vi "Glimpse Image Display Controller.vi"() -> ()   [LabVIEW 2015]
doc: "This widget allows the user to separately adjust the properties of mulltiple, independently displayed image windows. The controller is a stand-alone VI that can run in a separate thread from the program that is producing the images, so that the image display settings can be adjusted whilst other things (e.g., data acquisition) are occurring simultaneously."
uses:
  Image to Display event.ctt
  <vilib>/vision/Image Controls.llb/IMAQ Image.ctl
  GLIMPSE Globals.vi
panel:
  in  "to window":i8=9 min=2 max=9 step=1
  in  "Snapshot":bool
  in  "Presets":T1(array[cluster])=[{"Mem"=FALSE, "Black"=-32500.0, "White"=-25000.0, "Recall"=FALSE}]
  in  "Keep this in corner?":bool=TRUE
  in  "Autosize M":bool
  in  "Autoposition M":bool
  in  "Autoscale M":bool
  in  "Zoom +":bool
  in  "Zoom -":bool
  out "In use":bool
  in  "Auto size":bool
  in  "Auto position":bool
  in  "Autoscale":bool
  out "Window Title":string
  in  "Control image window #":u8(slide)=1 max=1 step=1 scale=0.0..1.0
  out "error out":errorcluster
  out "Black/White Levels temp":cluster{ext, ext}(slide)={1.0, 65535.0} scale=-32767.0..327567.0
  in  "Black/White Levels":cluster{ext, ext}(slide)={1.0, 65535.0} scale=-32767.0..327567.0
  in  "Stop":bool
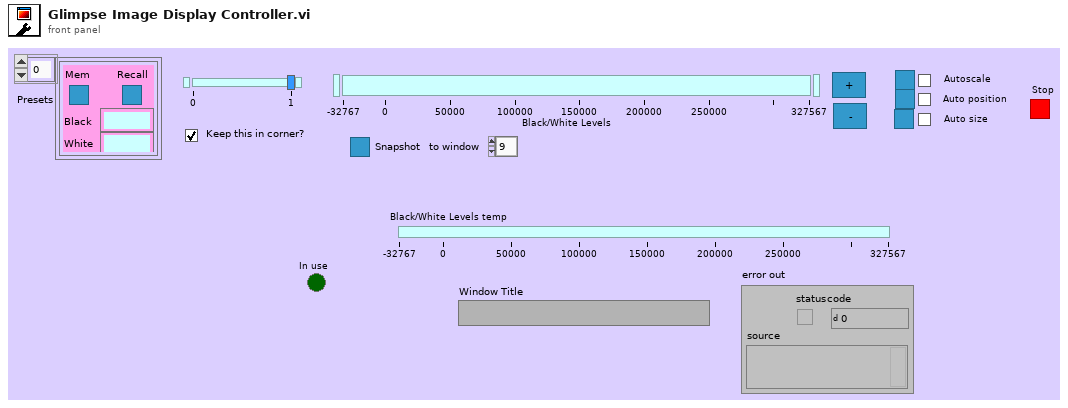
[diagram p1: front panel]
types:
  T1 = cluster{"Mem":bool, "Black":ext, "White":ext, "Recall":bool}[]
  T2 = typedef "Image Type" = u32
  T3 = typedef "IMAQ Image.ctl" = refnum<image>
  T4 = cluster{"Image Type":T2, "Image":T3, "Initialized?":bool, "Window Title":string, "Auto resize?":bool, "Auto position?":bool, "Autoscale?":bool, "Black/White Levels":cluster{ext, ext}, "Scale Min":ext, "Scale Max":ext}
  T5 = typedef "LVRectTypeDef.ctl" = cluster{"Left":i16, "Top":i16, "Right":i16, "Bottom":i16}
  T6 = typedef "Image to Display event.ctt" = cluster{"Image":T3, "Window Title":string, "Window Number":i32, "Image Type":T2, "Quit display controller?":bool}
  T7 = cluster{"Image Type":T2, "Image":T3, "Initialized?":bool, "Window Title":string, "Auto resize?":bool, "Auto position?":bool, "Autoscale?":bool, "Black/White Levels":cluster{ext, ext}, "Scale Min":ext, "Scale Max":ext}[]
  T8 = cluster{"Mem":bool, "Black":ext, "White":ext, "Recall":bool}
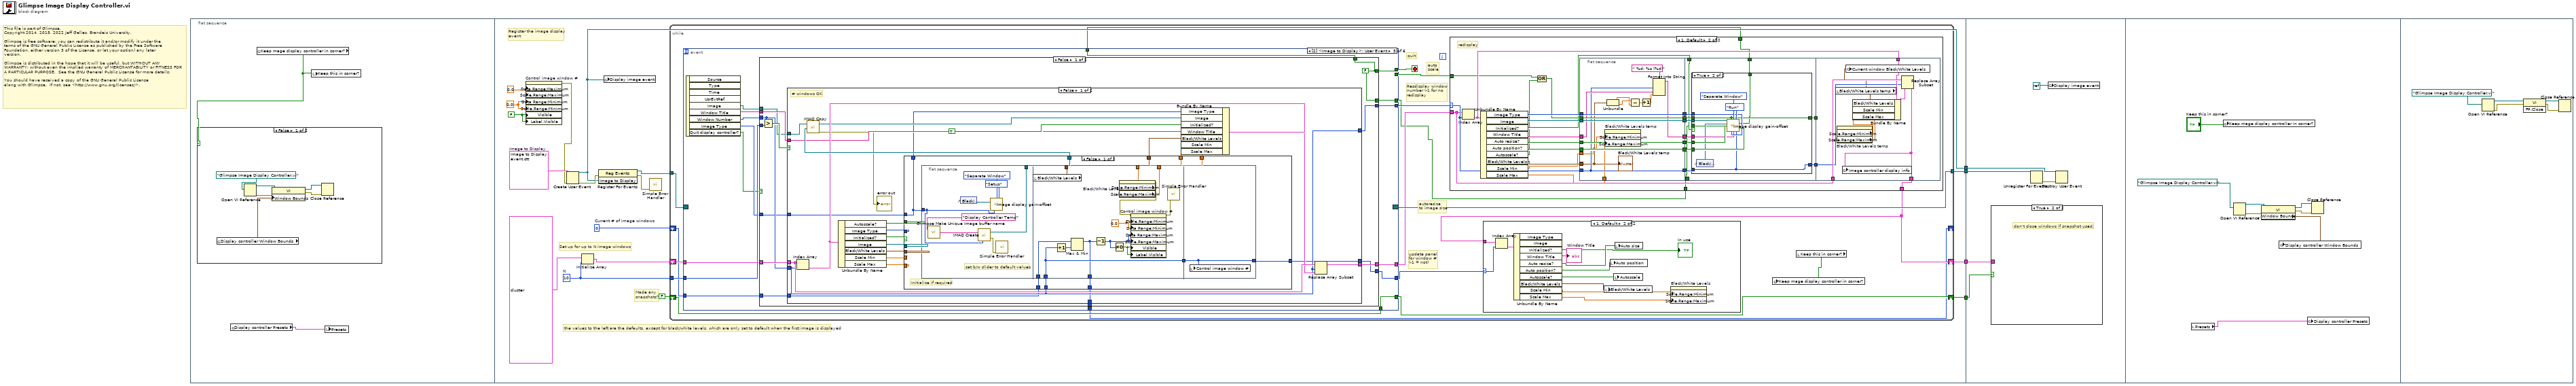
[diagram p0: block diagram]
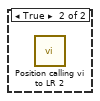
[diagram p2: hidden frame]
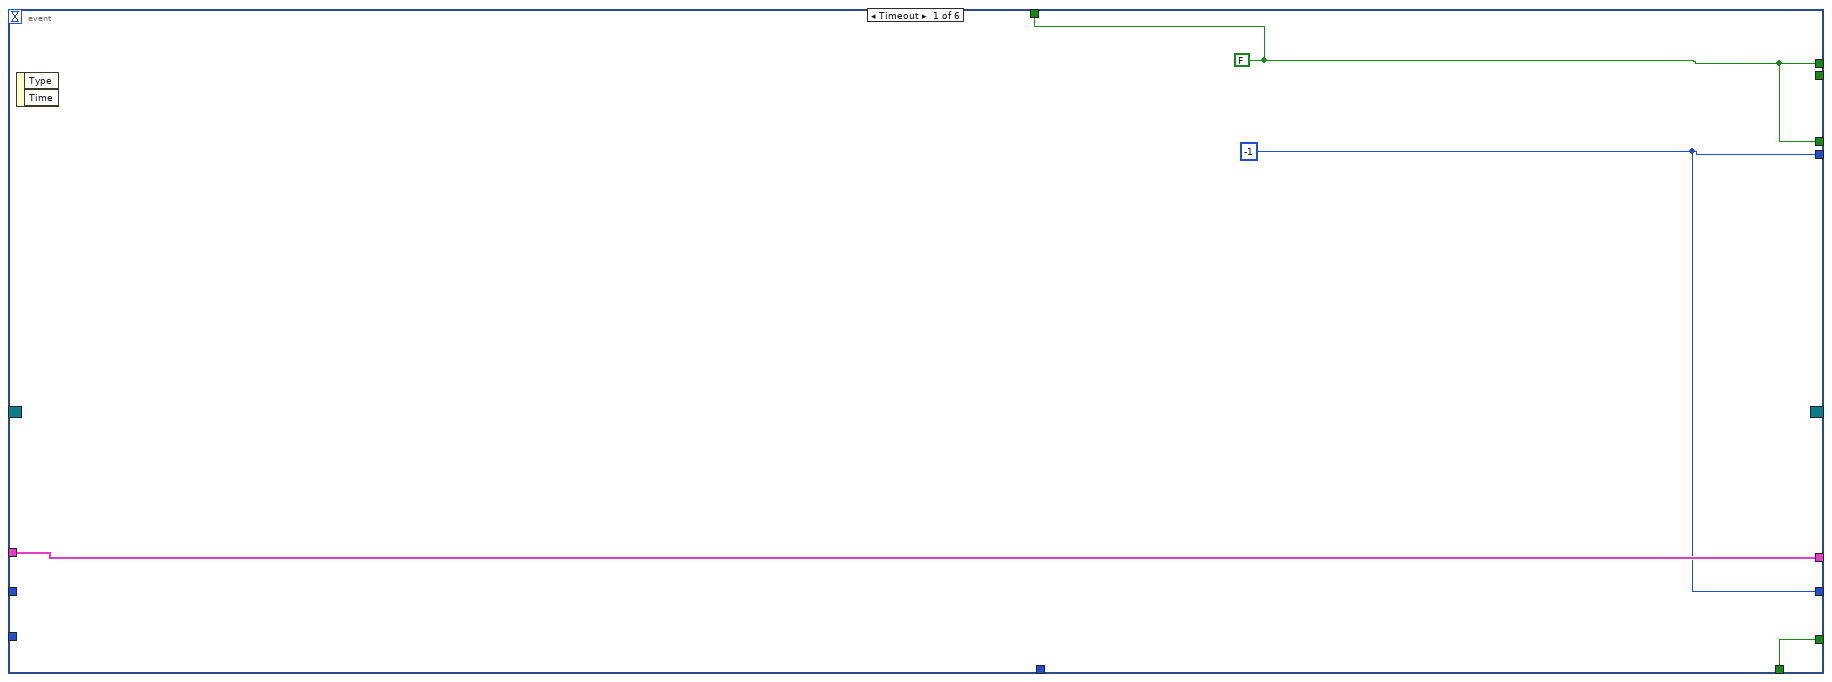
[diagram p6: hidden frame]
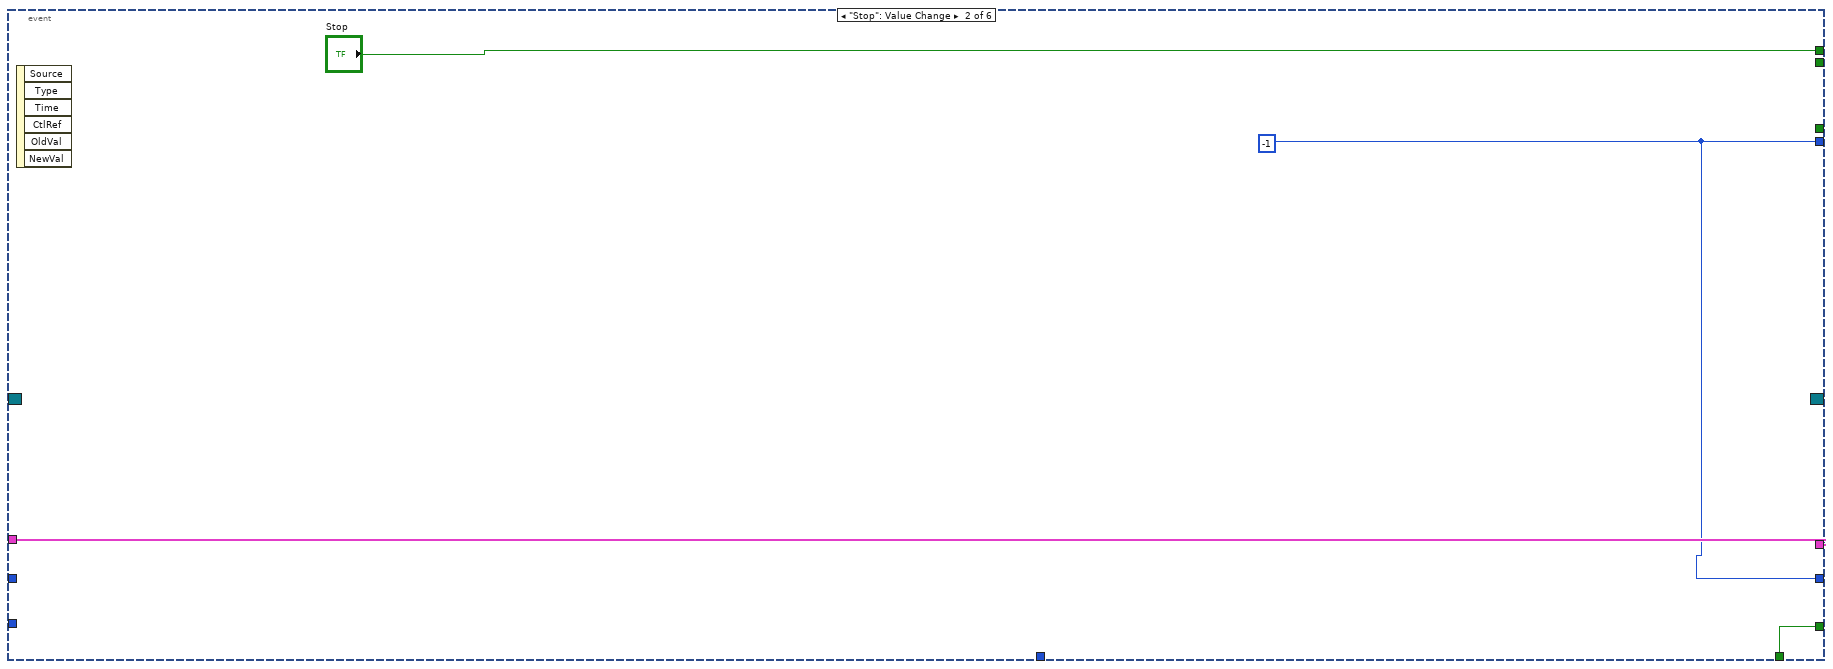
[diagram p7: hidden frame]
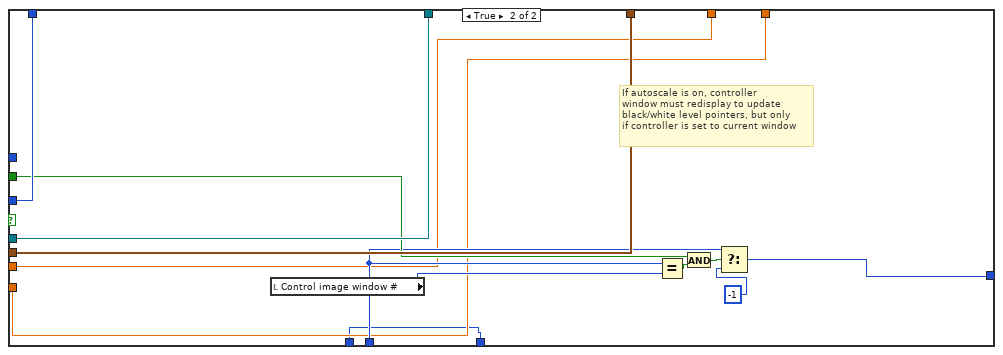
[diagram p8: hidden frame]
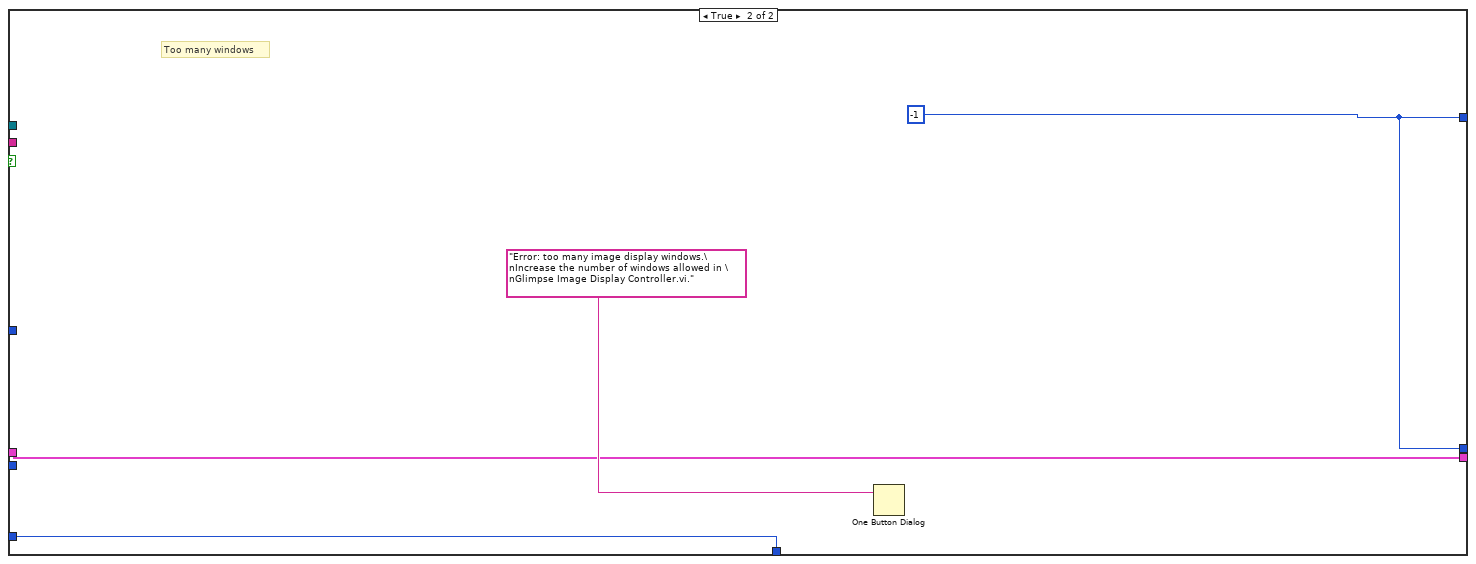
[diagram p9: hidden frame]
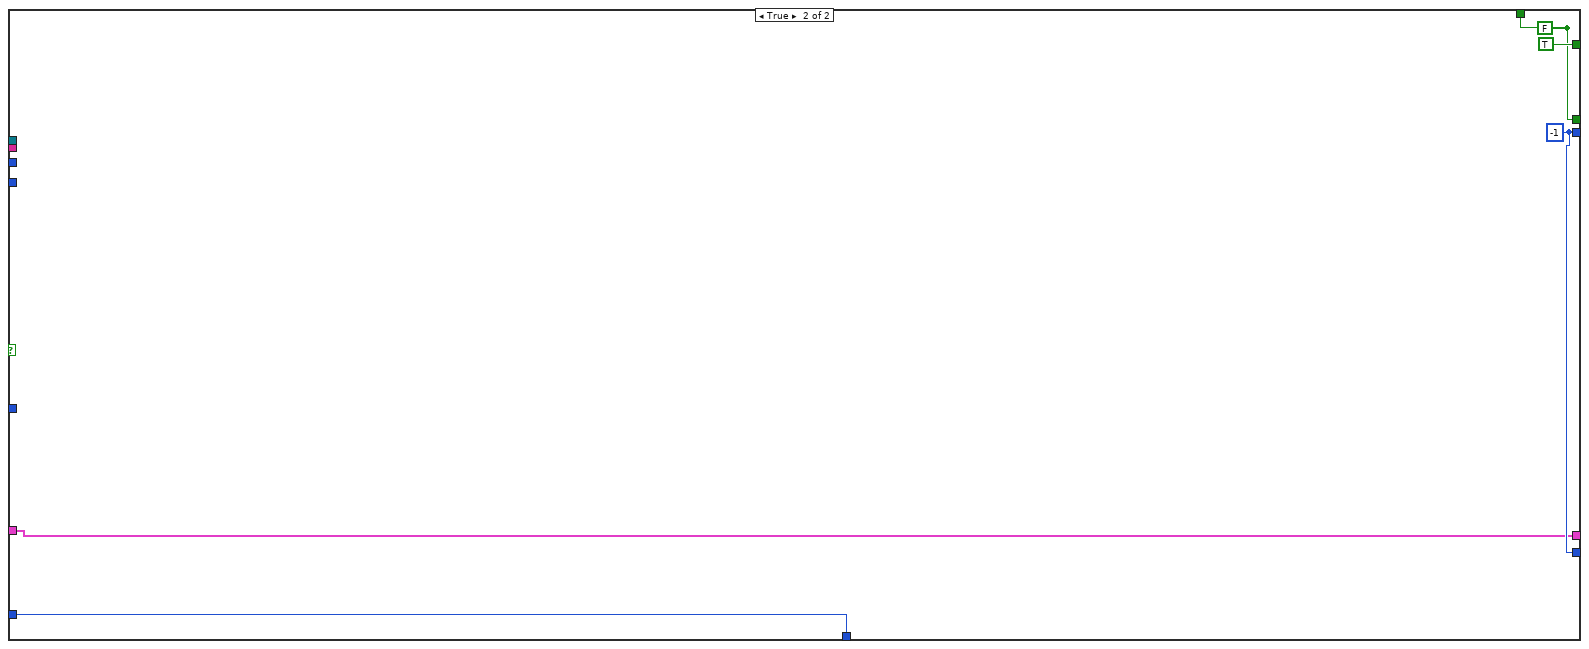
[diagram p10: hidden frame]
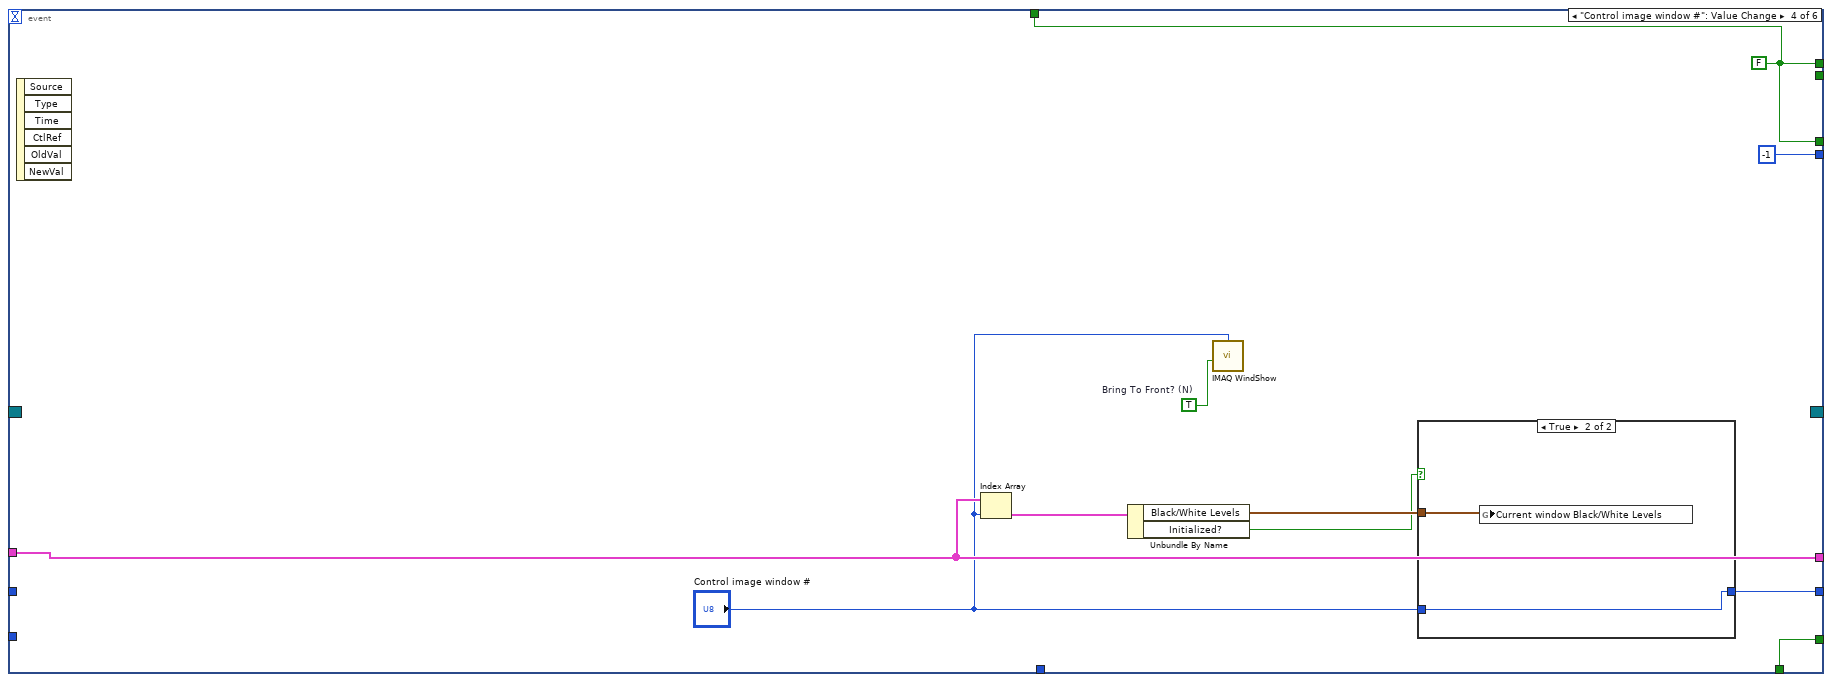
[diagram p11: hidden frame]
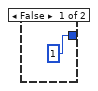
[diagram p12: hidden frame]
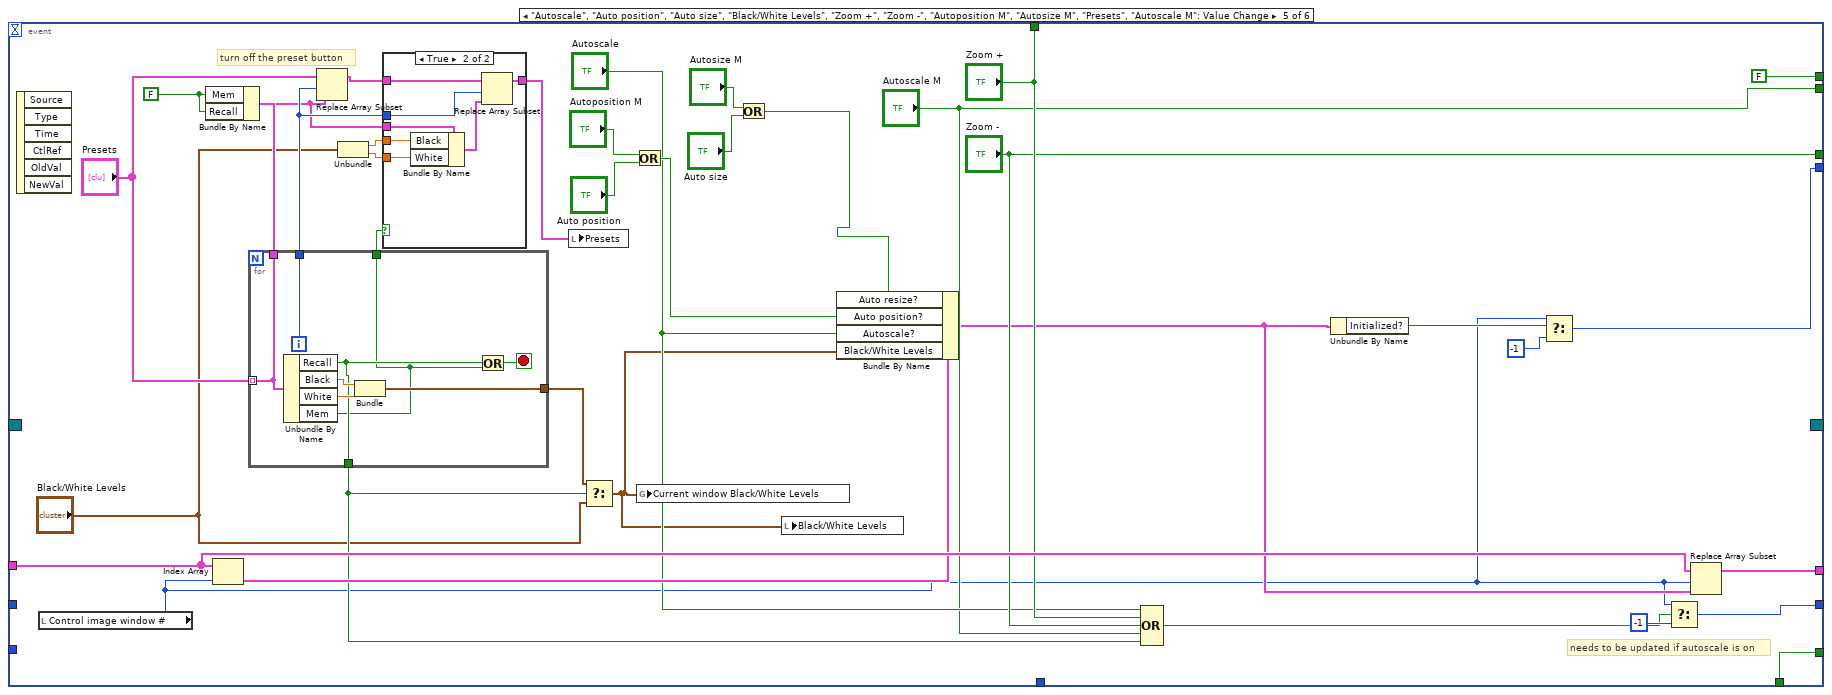
[diagram p13: hidden frame]
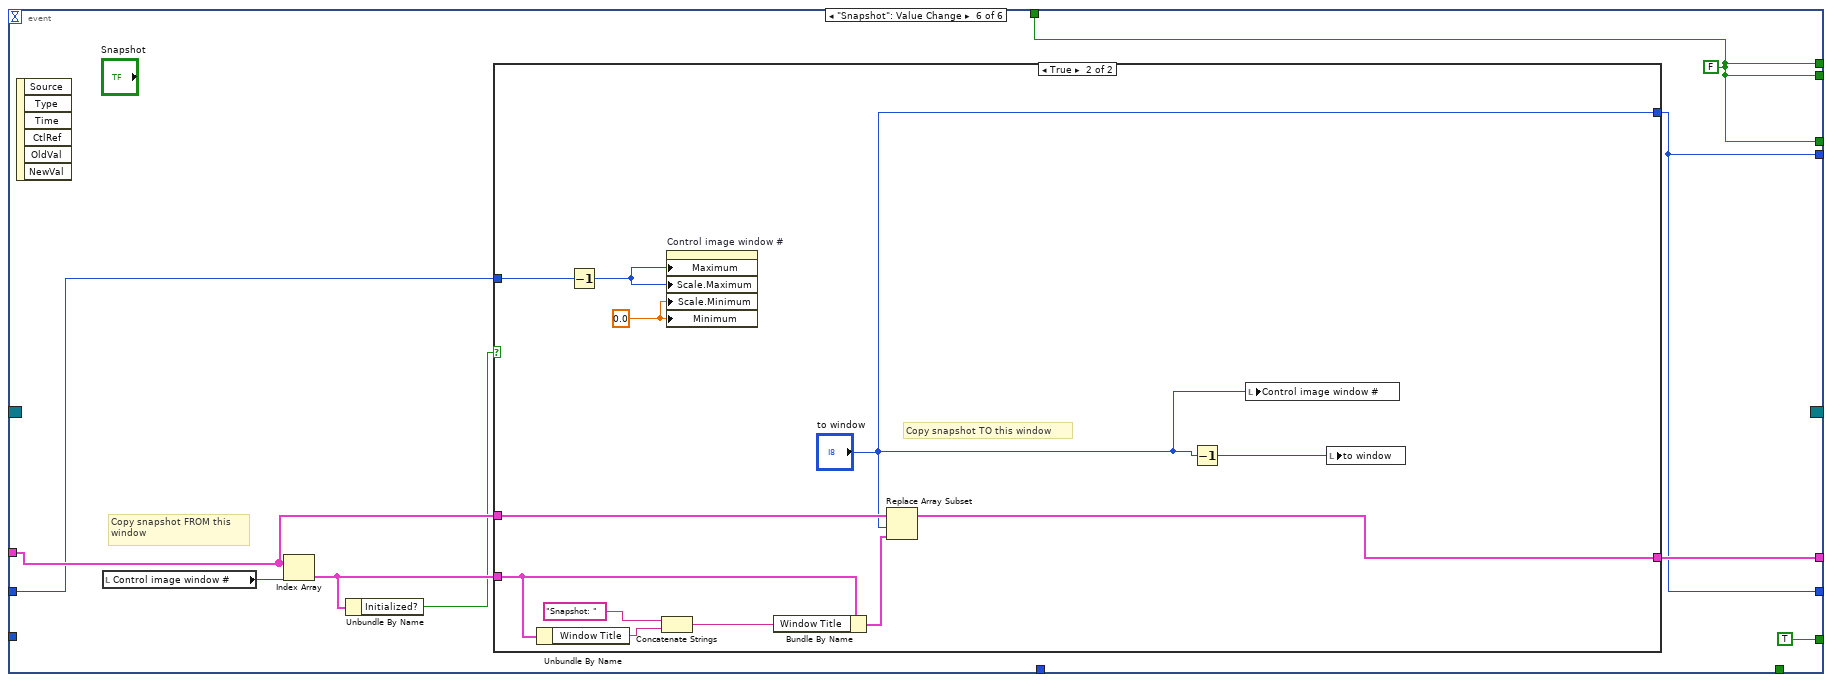
[diagram p15: hidden frame]
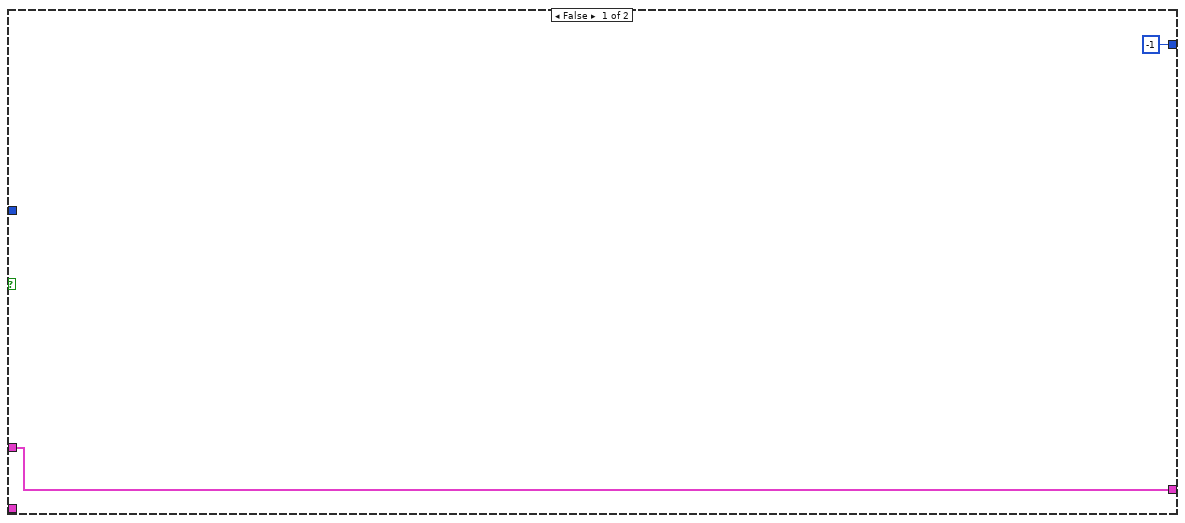
[diagram p16: hidden frame]
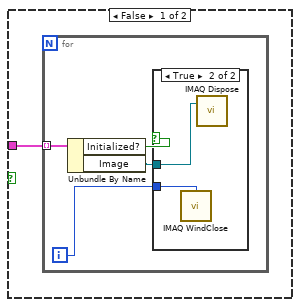
[diagram p17: hidden frame]
diagram:
  # "This file is part of Glimpse. \nCopyright 2014, 2015, 2022 Jeff Gelles, Brandeis University.    \n\nGlimpse is free software: you can redistribute it and/or modify it under the \nterms of the GNU General Public License as published by the Free Software \nFoundation, either version 3 of the License, or (at your option) any later \nversion.\n\nGlimpse is distributed in the hope that it will be useful, but WITHOUT ANY \nWARRANTY; without even the implied warranty of MERCHANTABILITY or FITNESS FOR \nA PARTICULAR PURPOSE.  See the GNU General Public License for more details.\n\nYou should have received a copy of the GNU General Public License\nalong with Glimpse.  If not, see <http://www.gnu.org/licenses/>."
  n1 = flat-sequence {
    tunnel: [w26] -> w4
    tunnel: [w20] -> w3
    tunnel: [w21] -> w2
    tunnel: [w16] -> w1
    tunnel: w4 -> [w346]
    tunnel: w3 -> [w344]
    tunnel: w2 -> [w342]
    tunnel: w1 -> [w341]
    frame #0 {
      n2 = global read "GLIMPSE Globals.vi" "Display controller Presets"() -> (w5:T1)
      n3 = global read "GLIMPSE Globals.vi" "Keep mage display controller in corner?"() -> (w6:bool)
      n4 = case shown="False" w6 {
        frame False {
          n5 = global read "GLIMPSE Globals.vi" "Display controller Window Bounds"() -> (w8:T5)
          n6 = Open VI Reference(vi path=path "Glimpse Image Display Controller.vi") -> (vi reference=w12:refnum<vi>, error out=w11:errorcluster)  [unwired: 2 in, 3 out]
          n7 = property class="VI"(reference=w12, error in=w11, "Front Panel Window:Window Bounds"=w8) -> (reference out=w10:refnum<vi>, error out=w9:errorcluster)
          n8 = Close Reference(reference=w10, error in (no error)=w9) -> ()  [unwired: 1 out]
        }
        frame True {
          n9 = call "Position calling vi to LR 2.vi"() -> ()  [unwired: 2 in, 4 out]
        }
      }
      n10 = local write "Keep this in corner?"(w6) -> ()
      n11 = local write "Presets"(w5) -> ()
    }
    frame #1 {
      w14 = 0  # Current # of image windows
      w13 = FALSE ("Visible")
      w18 = 0.0 ("Data Range:Maximum")
      w19 = 0.0 ("Data Range:Maximum")
      w22 = 10  # N
      w25 = T6 {"Image"=refnum, "Window Title"="", "Window Number"=0, "Image Type"=0, "Quit display controller?"=FALSE}  # Image to Display
      # "Made any \nsnapshots?"
      # "the values to the left are the defaults, except for black/white levels, which are only set to default when the first image is displayed"
      # "Set up for up to N image windows"
      # "Register the image display\nevent"
      n12 = property on="Control image window #" class="Slide (strict)"("Data Range:Maximum"=w19, "Scale.Range:Maximum"=w19, "Data Range:Minimum"=w18, "Scale.Range:Minimum"=w18, "Visible"=w13, "Label.Visible"=w13) -> (error out=w15:errorcluster)  [unwired: 2 in, 1 out]
      n13 = Create User Event(user event datatype=w25, error in=w15) -> (user event=w20:refnum<user-event>, error out=w28:errorcluster)
      n14 = Initialize Array(T4 {"Image Type"=0, "Image"=refnum, "Initialized?"=FALSE, "Window Title"="", "Auto resize?"=FALSE, "Auto position?"=FALSE, "Autoscale?"=FALSE, "Black/White Levels"={1.0, 2.0}, "Scale Min"=-32767.0, "Scale Max"=327567.0}, w22) -> (w23:T7)
      n15 = register-events(error in=w28, w20) -> (reference out=w29:refnum<event-registration>, error out=w27:errorcluster)  [unwired: 1 in]
      n16 = global write "GLIMPSE Globals.vi" "Display image event"(w20) -> ()
      n17 = call <vilib>:"Simple Error Handler.vi"("error in (no error)"=w27) -> ()  [unwired: 1 in, 8 out]
      n18 = while {
        shift-right: [w39] -> w21
        shift-left: w23 -> [w44]
        tunnel: w29 -> [w45]
        tunnel: [w41] -> w26
        tunnel: w22 -> [w43]
        shift-right: [w33] -> w16
        shift-left: FALSE ("Stop") -> [w32]
        shift-right: [w30] -> _
        shift-left: w14 -> [w31]
        stop <- w46 stop-if-true
        # "autoresize\nto image size"
        # "auto\nscale"
        # "update panel\nfor window #\n(-1 = not)"
        # "quit"
        # "Resdisplay window\nnumber (-1 for no\nredisplay"
        n19 = event shown="[2] <Image to Display>: User Event" {
          selector: w45 -> [_ _ _ _ _ _]
          dyn-events: [_ _ _ _ _ _] -> w41
          timeout: _ -> [_ _ _ _ _ _]
          tunnel: [w138 "Stop" w154 w257 FALSE ("Stop") w324] -> w46
          tunnel: w44 -> [w139 w142 w158 w260 w301 w326]
          tunnel: w43 -> [_ _ w159 _ _ w323]
          tunnel: [w139 w142 w155 w260 w294 w325] -> w40
          tunnel: [w137 w141 w151 -1 ("Window Number") w268 w319] -> w42
          tunnel: [w138 _ w148 w257 "Zoom +" w324] -> w38
          tunnel: [w138 _ w149 w257 "Zoom -" w324] -> w35
          tunnel: [_ _ _ _ "Autoscale M" w324] -> w37
          tunnel: [w137 w141 w147 w253 w271 w319] -> w34
          tunnel: [w136 w140 w146 w252 w265 TRUE ("Stop")] -> w33
          tunnel: w32 -> [w136 w140 w146 w252 w265 _]
          tunnel: w31 -> [_ _ w145 _ _ _]
          tunnel: [_ _ w144 _ _ _] -> w30
          event Timeout {
            w137 = -1 ("Window Number")
            w138 = FALSE ("Stop")
            n20 = event-data() -> ()  [unwired: 3 out]
          }
          event "Stop": Value Change {
            w141 = -1 ("Window Number")
            n21 = event-data() -> ()  [unwired: 7 out]
          }
          event User Event {
            n22 = event-data() -> ("Image"=w152:T3, "Window Title"=w156:string, "Window Number"=w157:i32, "Image Type"=w153:T2, "Quit display controller?"=w150:bool)  [unwired: 5 out]
            n23 = case shown="False" w150 {
              tunnel: w159 -> [w172 _]
              tunnel: w158 -> [w170 w249]
              tunnel: w157 -> [w169 _]
              tunnel: w156 -> [w168 _]
              tunnel: [w167 w249] -> w155
              tunnel: [w162 TRUE] -> w154
              tunnel: w153 -> [w166 _]
              tunnel: w152 -> [w165 _]
              tunnel: [w164 w250] -> w151
              tunnel: [w163 w250] -> w147
              tunnel: [w162 w248] -> w149
              tunnel: [w162 w248] -> w148
              tunnel: w145 -> [w161 w247]
              tunnel: [w160 w247] -> w144
              frame False {
                w162 = FALSE
                n24 = Greater?(x=w169, y=w172) -> (0:w171:bool)
                n25 = case shown="False" w171 {
                  tunnel: w170 -> [w189 w245]
                  tunnel: w169 -> [w183 _]
                  tunnel: w165 -> [w195 _]
                  tunnel: w168 -> [w190 _]
                  tunnel: [w175 w245] -> w167
                  tunnel: [w183 w244] -> w164
                  tunnel: w166 -> [w186 _]
                  tunnel: [w182 w244] -> w163
                  tunnel: w161 -> [w174 w243]
                  tunnel: [w173 w243] -> w160
                  frame False {
                    # "# windows OK"
                    n26 = Index Array(array=w189, index=w183) -> (element=w194:T4)
                    n27 = Unbundle By Name(w194) -> ("Autoscale?"=w180:bool, "Image Type"=w191:T2, "Initialized?"=w198:bool, "Image"=w197:T3, "Black/White Levels"=w184:cluster{ext, ext}, "Scale Min"=w177:ext, "Scale Max"=w176:ext)
                    n28 = case shown="False" w198 {
                      tunnel: w191 -> [_ w241]
                      tunnel: [w208 w242] -> w196
                      tunnel: w197 -> [_ w242]
                      tunnel: [w207 w241] -> w187
                      tunnel: w186 -> [w207 _]
                      tunnel: w184 -> [_ w240]
                      tunnel: [w206 w240] -> w181
                      tunnel: w183 -> [w205 w233]
                      tunnel: [w204 w237] -> w182
                      tunnel: w180 -> [_ w238]
                      tunnel: [w203 w232] -> w179
                      tunnel: [w202 w231] -> w178
                      tunnel: w177 -> [_ w232]
                      tunnel: w176 -> [_ w231]
                      tunnel: w174 -> [w200 w230]
                      tunnel: [w199 w230] -> w173
                      frame False {
                        # "Initialize if required"
                        n29 = flat-sequence {
                          tunnel: [w214] -> w208
                          tunnel: w207 -> [w209]
                          tunnel: [w228] -> w206
                          tunnel: w205 -> [w225]
                          tunnel: [w227] -> w203
                          tunnel: [w226] -> w202
                          tunnel: [w225] -> w201
                          tunnel: w200 -> [w221]
                          tunnel: [w219] -> w199
                          tunnel: [w229] -> w204
                          tunnel: w201 -> [w229]
                          frame #0 {
                            # "set b/w slider to default values"
                            n30 = call "Glimpse Make Unique Image buffer name.vi"("Buffer  base name"="Display Controller Temp") -> ("Image Name"=w215:string)  [unwired: 1 out]
                            n31 = control-ref of="Black/White Levels"() -> (w210:refnum<vi>)
                            n32 = call "IMAQ Create"("Image Name"=w215, "Image Type"=w209) -> ("New Image"=w214:T3, "error out"=w213:errorcluster)  [unwired: 2 in, 1 out]
                            n33 = call "Image display gain-offset.vi"("Display Type (s)"=enum16{"Front Panel", "Separate Window"}."Separate Window", "Mode"=enum16{"Setup", "Run"}."Setup", "Black/White Levels Ctl Ref (s)"=w210, "Pixel depth (s)"=w209) -> ()  [unwired: 9 in, 3 out]
                            n34 = call <vilib>:"Simple Error Handler.vi"("error in (no error)"=w213) -> ()  [unwired: 1 in, 8 out]
                          }
                          frame #1 {
                            w223 = 0.0 ("Data Range:Minimum")
                            n35 = local read "Black/White Levels"() -> (w228:cluster{ext, ext})
                            n36 = Increment(x=w225) -> (x+1=w220:i32)
                            n37 = Max & Min(x=w221, y=w220) -> (max(x,y)=w219:i32)  [unwired: 1 out]
                            n38 = Decrement(x=w219) -> (x-1=w218:i32)
                            n39 = Not Equal To 0?(x=w218) -> (x != 0?=w217:bool)
                            n40 = property on="Black/White Levels" class="Slide (strict)"() -> (error out=w222:errorcluster, "Scale.Range:Minimum"=w227:dbl, "Scale.Range:Maximum"=w226:dbl)  [unwired: 2 in, 1 out]
                            n41 = property on="Control image window #" class="Slide (strict)"(error in=w222, "Scale.Range:Minimum"=w223, "Data Range:Minimum"=w223, "Data Range:Maximum"=w218, "Scale.Range:Maximum"=w218, "Visible"=w217, "Label.Visible"=w217) -> (error out=w224:errorcluster)  [unwired: 1 in, 1 out]
                            n42 = call <vilib>:"Simple Error Handler.vi"("error in (no error)"=w224) -> ()  [unwired: 1 in, 8 out]
                          }
                          frame #2 {
                            n43 = local write "Control image window #"(w229) -> ()
                          }
                        }
                      }
                      frame True {
                        # "If autoscale is on, controller\nwindow must redisplay to update \nblack/white level pointers, but only\nif controller is set to current window"
                        n44 = local read "Control image window #"() -> (w234:u8)
                        n45 = Equal?(x=w233, y=w234) -> (x = y?=w235:bool)
                        n46 = And(x=w238, y=w235) -> (x .and. y?=w236:bool)
                        n47 = Select(t=w233, s=w236, f=-1 ("Window Number")) -> (s? t:f=w237:i32)
                      }
                    }
                    n48 = call "IMAQ Copy"("Image Dst"=w196, "Image Src"=w195) -> ("error out"=→"error out":errorcluster, "Image Dst Out"=w193:T3)  [unwired: 1 in, 3 out]
                    n49 = Bundle By Name(cluster=w194, "Image Type"=w187, "Image"=w193, "Initialized?"=TRUE, "Window Title"=w190, "Black/White Levels"=w181, "Scale Min"=w179, "Scale Max"=w178) -> (w188:T4)
                    n50 = Replace Array Subset(array=w189, new element=w188, index=w183) -> (w175:T7)
                  }
                  frame True {
                    w244 = -1 ("Window Number")
                    # "Too many windows"
                    n51 = One Button Dialog(message="Error: too many image display windows.\nIncrease the number of windows allowed in \nGlimpse Image Display Controller.vi.") -> ()  [unwired: 2 out]
                  }
                }
              }
              frame True {
                w248 = FALSE
                w250 = -1 ("Window Number")
              }
            }
          }
          event "Control image window #": Value Change {
            w256 = TRUE  # Bring To Front? (N)
            w257 = FALSE ("Stop")
            n52 = event-data() -> ()  [unwired: 7 out]
            n53 = Index Array(array=w260, index="Control image window #") -> (element=w259:T4)
            n54 = Unbundle By Name(w259) -> ("Black/White Levels"=w258:cluster{ext, ext}, "Initialized?"=w255:bool)
            n55 = call "IMAQ WindShow"("Bring To Front? (N)"=w256, "Window Number (0...15)"="Control image window #") -> ()  [unwired: 3 in, 4 out]
            n56 = case shown="True" w255 {
              tunnel: w258 -> [_ w264]
              tunnel: "Control image window #" -> [_ w263]
              tunnel: [i8 1 ("Control image window #") w263] -> w253
              frame False {
              }
              frame True {
                n57 = global write "GLIMPSE Globals.vi" "Current window Black/White Levels"(w264) -> ()
              }
            }
          }
          event "Autoscale", "Auto position", "Auto size", "Black/White Levels", "Zoom +", "Zoom -", "Autoposition M", "Autosize M", "Presets", "Autoscale M": Value Change {
            w281 = FALSE ("Select")
            # "turn off the preset button"
            # "needs to be updated if autoscale is on"
            n58 = event-data() -> ()  [unwired: 7 out]
            n59 = local read "Control image window #"() -> (w266:u8)
            n60 = Index Array(array=w301, index=w266) -> (element=w300:T4)
            n61 = for {
              tunnel: "Presets" -> [w313] mode=indexing
              tunnel: [w315] -> w285
              tunnel: [w311] -> w282
              tunnel: [w314] -> w278
              tunnel: [w313] -> w284
              tunnel: [w310] -> w277
              i -> [w314]
              stop <- w312 stop-if-true
              n62 = Unbundle By Name(w313) -> ("Recall"=w311:bool, "Black"=w317:ext, "White"=w316:ext, "Mem"=w310:bool)
              n63 = Bundle("Black"=w317, "White"=w316) -> (w315:cluster{"Black":ext, "White":ext})  [unwired: 1 out]
              n64 = Or(x=w311, y=w310) -> (x .or. y?=w312:bool)
            }
            n65 = Bundle By Name(cluster=w284, "Mem"=w281, "Recall"=w281) -> (w276:T8)
            n66 = Replace Array Subset(array="Presets", new element=w276, index=w278) -> (w280:T1)
            n67 = Unbundle("Black/White Levels") -> (w273:ext, w274:ext)
            n68 = case shown="True" w277 {
              tunnel: w280 -> [w302 w309]
              tunnel: [w302 w308] -> w279
              tunnel: w278 -> [_ w307]
              tunnel: w276 -> [_ w306]
              tunnel: w274 -> [_ w304]
              tunnel: w273 -> [_ w303]
              frame False {
              }
              frame True {
                n69 = Bundle By Name(cluster=w306, "Black"=w303, "White"=w304) -> (w305:T8)
                n70 = Replace Array Subset(array=w309, new element=w305, index=w307) -> (w308:T1)
              }
            }
            n71 = local write "Presets"(w279) -> ()
            n72 = Select(t=w285, s=w282, f="Black/White Levels") -> (s? t:f=w272:cluster{"Black":ext, "White":ext})
            n73 = Or(x="Autoposition M", y="Auto position") -> (x .or. y?=w292:bool)
            n74 = global write "GLIMPSE Globals.vi" "Current window Black/White Levels"(w272) -> ()
            n75 = Or(x="Autosize M", y="Auto size") -> (x .or. y?=w290:bool)
            n76 = local write "Black/White Levels"(w272) -> ()
            n77 = Bundle By Name(cluster=w300, "Auto resize?"=w290, "Auto position?"=w292, "Autoscale?"="Autoscale", "Black/White Levels"=w272) -> (w270:T4)
            n78 = Compound Arithmetic op=OR("Autoscale", "Zoom +", "Zoom -", "Autoscale M", w282) -> (w297:bool)
            n79 = Unbundle By Name(w270) -> ("Initialized?"=w269:bool)
            n80 = Select(t=w266, s=w269, f=-1 ("s? t:f")) -> (s? t:f=w268:i32)
            n81 = Select(t=w266, s=w297, f=-1) -> (s? t:f=w271:i32)
            n82 = Replace Array Subset(array=w301, new element=w270, index=w266) -> (w294:T7)
          }
          event "Snapshot": Value Change {
            w324 = FALSE ("Stop")
            # "Copy snapshot FROM this\nwindow"
            n83 = event-data() -> ()  [unwired: 7 out]
            n84 = local read "Control image window #"() -> (w322:u8)
            n85 = Index Array(array=w326, index=w322) -> (element=w321:T4)
            n86 = Unbundle By Name(w321) -> ("Initialized?"=w320:bool)
            n87 = case shown="True" w320 {
              tunnel: w326 -> [w328 w340]
              tunnel: [w328 w339] -> w325
              tunnel: [i8 -1 ("to window") "to window"] -> w319
              tunnel: w323 -> [_ w333]
              tunnel: w321 -> [_ w330]
              frame False {
              }
              frame True {
                w332 = 0.0 ("Data Entry Limits:Minimum")
                # "Copy snapshot TO this window"
                n88 = Unbundle By Name(w330) -> ("Window Title"=w336:string)
                n89 = Decrement(x=w333) -> (x-1=w331:i32)
                n90 = Concatenate Strings("Snapshot: " ("string"), w336) -> (w335:string)
                n91 = property on="Control image window #" class="Slide (strict)"("Maximum"=w331, "Scale.Maximum"=w331, "Scale.Minimum"=w332, "Minimum"=w332) -> ()  [unwired: 2 in, 2 out]
                n92 = Bundle By Name(cluster=w330, "Window Title"=w335) -> (w334:T4)
                n93 = Replace Array Subset(array=w340, new element=w334, index="to window") -> (w339:T7)
                n94 = Decrement(x="to window") -> (x-1=w329:i8)
                n95 = local write "Control image window #"("to window") -> ()
                n96 = local write "to window"(w329) -> ()
              }
            }
          }
        }
        n97 = case shown="1, Default" w42 {
          selector: w42 -> [_ w82]
          tunnel: w40 -> [w58 w70]
          tunnel: [w58 w67] -> w39
          tunnel: w38 -> [_ w63]
          tunnel: w37 -> [_ w60]
          tunnel: w35 -> [_ w59]
          frame -1 {
          }
          frame 1, Default {
            # "redisplay"
            n98 = Index Array(array=w70, index=w82) -> (element=w68:T4)
            n99 = Unbundle By Name(w68) -> ("Image Type"=w83:T2, "Image"=w85:T3, "Initialized?"=w71:bool, "Window Title"=w81:string, "Auto resize?"=w84:bool, "Auto position?"=w80:bool, "Autoscale?"=w61:bool, "Black/White Levels"=w72:cluster{ext, ext}, "Scale Min"=w65:ext, "Scale Max"=w64:ext)
            n100 = Or(x=w60, y=w61) -> (x .or. y?=w62:bool)
            n101 = flat-sequence {
              tunnel: w80 -> [w97]
              tunnel: w81 -> [w95]
              tunnel: w82 -> [w93]
              tunnel: w83 -> [w98]
              tunnel: w84 -> [w99]
              tunnel: w85 -> [w100]
              tunnel: w62 -> [w101]
              tunnel: [w101] -> w79
              tunnel: [w100] -> w78
              tunnel: [w99] -> w77
              tunnel: [w98] -> w76
              tunnel: [w93] -> w75
              tunnel: [w94] -> w74
              tunnel: [w97] -> w73
              tunnel: w72 -> [w92]
              tunnel: w65 -> [w87]
              tunnel: w64 -> [w86]
              tunnel: w79 -> [w113]
              tunnel: w78 -> [w112]
              tunnel: w77 -> [w111]
              tunnel: w76 -> [w110]
              tunnel: w75 -> [w109]
              tunnel: w74 -> [w108]
              tunnel: w73 -> [w107]
              tunnel: w71 -> [w106]
              tunnel: [w105] -> w69
              tunnel: [w104] -> w66
              tunnel: w63 -> [w103]
              tunnel: w59 -> [w102]
              tunnel: w70 -> [w135]
              tunnel: w69 -> [w133]
              tunnel: w68 -> [w134]
              tunnel: [w129] -> w67
              tunnel: w66 -> [_]
              frame #0 {
                n102 = property on="Black/White Levels temp" class="Slide (strict)"("Scale.Range:Minimum"=w87, "Scale.Range:Maximum"=w86) -> ()  [unwired: 2 in, 2 out]
                n103 = Unbundle(w92) -> (w90:ext, w91:ext)
                n104 = Subtract(x=w91, y=w90) -> (x-y=w89:ext)
                n105 = Increment(x=w89) -> (x+1=w88:ext)
                n106 = Format Into String(format string=" %d: %s (%d)", w93, w95, w88) -> (resulting string=w94:string)  [unwired: 2 in, 1 out]
                "Black/White Levels temp" <- w92
              }
              frame #1 {
                n107 = case shown="True" w106 {
                  tunnel: w113 -> [w114 w119]
                  tunnel: w112 -> [_ w125]
                  tunnel: w111 -> [_ w124]
                  tunnel: w110 -> [_ w123]
                  tunnel: w109 -> [w115 w116]
                  tunnel: w108 -> [_ w122]
                  tunnel: w107 -> [_ w121]
                  tunnel: [w115 w116] -> w105
                  tunnel: [w114 w119] -> w104
                  tunnel: w103 -> [_ w118]
                  tunnel: w102 -> [_ w117]
                  frame False {
                  }
                  frame True {
                    n108 = control-ref of="Black/White Levels temp"() -> (w120:refnum<vi>)
                    n109 = call "Image display gain-offset.vi"("Image In"=w125, "Autoscale?"=w119, "Display Type (s)"=enum16{"Front Panel", "Separate Window"}."Separate Window", "Mode"=enum16{"Setup", "Run"}."Run", "Black/White Levels Ctl Ref (s)"=w120, "Zoom +"=w118, "Auto Resize to Image Size?\n(Window only)"=w124, "Zoom -"=w117, "Auto position\n(Window only)"=w121, "Pixel depth (s)"=w123, "Window Title\n(Window only)"=w122, "Window Number\n(Window only)"=w116) -> ()  [unwired: 1 in, 3 out]
                  }
                }
              }
              frame #2 {
                n110 = local read "Black/White Levels temp"() -> (w128:cluster{ext, ext})
                n111 = property on="Black/White Levels temp" class="Slide (strict)"() -> ("Scale.Range:Minimum"=w131:dbl, "Scale.Range:Maximum"=w130:dbl)  [unwired: 2 in, 2 out]
                n112 = global write "GLIMPSE Globals.vi" "Current window Black/White Levels"(w128) -> ()
                n113 = Bundle By Name(cluster=w134, "Black/White Levels"=w128, "Scale Min"=w131, "Scale Max"=w130) -> (w132:T4)
                n114 = Replace Array Subset(array=w135, new element=w132, index=w133) -> (w129:T7)
                n115 = global write "GLIMPSE Globals.vi" "Image controller display info"(w129) -> ()
              }
            }
          }
        }
        n116 = case shown="1, Default" w34 {
          selector: w34 -> [_ w50]
          tunnel: w39 -> [_ w56]
          frame -1 {
          }
          frame 1, Default {
            n117 = Index Array(array=w56, index=w50) -> (element=w57:T4)
            n118 = Unbundle By Name(w57) -> ("Initialized?"=→"In use":bool, "Window Title"=→"Window Title":string, "Auto resize?"=w53:bool, "Auto position?"=w52:bool, "Autoscale?"=w51:bool, "Black/White Levels"=w54:cluster{ext, ext}, "Scale Min"=w47:ext, "Scale Max"=w48:ext)  [unwired: 2 out]
            n119 = local write "Black/White Levels"(w54) -> ()
            n120 = local write "Auto position"(w52) -> ()
            n121 = local write "Autoscale"(w51) -> ()
            n122 = local write "Auto size"(w53) -> ()
            n123 = property on="Black/White Levels" class="Slide (strict)"("Scale.Range:Minimum"=w47, "Scale.Range:Maximum"=w48) -> ()  [unwired: 2 in, 2 out]
          }
        }
        n124 = local read "Keep this in corner?"() -> (w36:bool)
        n125 = global write "GLIMPSE Globals.vi" "Keep mage display controller in corner?"(w36) -> ()
      }
    }
    frame #2 {
      n126 = case shown="True" w341 {
        tunnel: w342 -> [w347 _]
        frame False {
          n127 = for {
            tunnel: w347 -> [w351] mode=indexing
            i -> [w348]
            n128 = Unbundle By Name(w351) -> ("Initialized?"=w350:bool, "Image"=w349:T3)
            n129 = case shown="True" w350 {
              tunnel: w349 -> [_ w353]
              tunnel: w348 -> [_ w352]
              frame False {
              }
              frame True {
                n130 = call "IMAQ WindClose"("Window Number (0...15)"=w352) -> ()  [unwired: 2 in, 4 out]
                n131 = call "IMAQ Dispose"("Image"=w353) -> ()  [unwired: 2 in, 4 out]
              }
            }
          }
        }
        frame True {
          # "don't close windows if snapshot used."
        }
      }
      n132 = Unregister For Events(event registration refnum=w346) -> (error out=w345:errorcluster)  [unwired: 1 in]
      n133 = global write "GLIMPSE Globals.vi" "Display image event"(refnum<k0> refnum) -> ()
      n134 = Destroy User Event(user event=w344, error in=w345) -> ()  [unwired: 1 out]
    }
    frame #3 {
      n135 = local read "Presets"() -> (w354:T1)
      n136 = global write "GLIMPSE Globals.vi" "Keep mage display controller in corner?"("Keep this in corner?") -> ()
      n137 = Open VI Reference(vi path=path "Glimpse Image Display Controller.vi") -> (vi reference=w360:refnum<vi>, error out=w359:errorcluster)  [unwired: 1 in, 4 out]
      n138 = property class="VI"(reference=w360, error in=w359) -> (reference out=w358:refnum<vi>, error out=w357:errorcluster, "Front Panel Window:Window Bounds"=w356:T5)
      n139 = global write "GLIMPSE Globals.vi" "Display controller Window Bounds"(w356) -> ()
      n140 = global write "GLIMPSE Globals.vi" "Display controller Presets"(w354) -> ()
      n141 = Close Reference(reference=w358, error in (no error)=w357) -> ()  [unwired: 1 out]
    }
    frame #4 {
      n142 = Open VI Reference(vi path=path "Glimpse Image Display Controller.vi") -> (vi reference=w363:refnum<vi>, error out=w364:errorcluster)  [unwired: 1 in, 4 out]
      n143 = invoke class="VI" method="FP.Close"(reference=w363, error in=w364) -> (reference out=w365:refnum<vi>, error out=w366:errorcluster)  [unwired: 1 in, 1 out]
      n144 = Close Reference(reference=w365, error in (no error)=w366) -> ()  [unwired: 1 out]
    }
  }
